vi "Test Read Linker Info.vi"(8 "error in (no error)":errorcluster) -> (0 "error out":errorcluster)   [LabVIEW 2020]
uses:
  classes/Test Runner.Folder/Test Runner.Folder.lvclass
  C:/projects/caraya/src/classes/Test Runner/Test Runner.lvclass
  classes/Test/Test.lvclass
  classes/Assert/Assert.lvclass
  classes/Test Runner/Test Runner.lvclass
panel:
  out "Test VIs":path[](array[path])
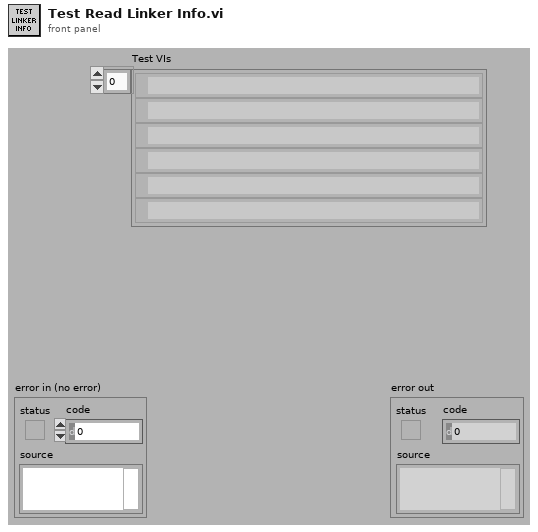
[diagram p1: front panel]
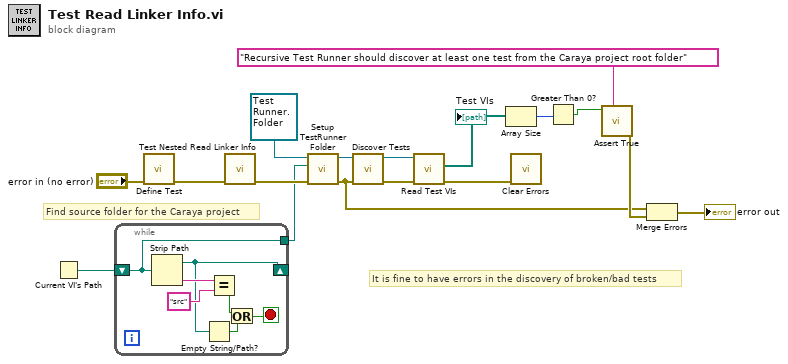
[diagram p0: block diagram]
diagram:
  # "It is fine to have errors in the discovery of broken/bad tests"
  # "Find source folder for the Caraya project"
  n1 = Current VI's Path() -> (path=w7:path)
  n2 = while {
    shift-right: [w18] -> _
    shift-left: w7 -> [w22]
    tunnel: [w22] -> w6
    stop <- w20 stop-if-true
    n3 = Strip Path(path=w22) -> (stripped path=w18:path, name=w24:string)
    n4 = Empty String/Path?(string/path=w18) -> (empty?=w19:bool)
    n5 = Equal?(x=w24, y="src") -> (x = y?=w21:bool)
    n6 = Or(x=w21, y=w19) -> (x .or. y?=w20:bool)
  }
  n7 = call "Define Test.vi"("error in (no error)"="error in (no error)") -> ("error out"=w16:errorcluster)  [unwired: 9 in, 1 out]
  n8 = call "Test Nested Read Linker Info.vi"("error in (no error)"=w16) -> ("error out"=w10:errorcluster)  [unwired: 10 in]
  n9 = call "Setup TestRunner Folder.vi"("error in (no error)"=w10, "Directory to search"=w6, "Test Runner.Folder"=refnum<class "Test Runner.Folder.lvclass"> refnum ("Caraya.lvlib:Test Runner.Folder.lvclass")) -> ("error out"=w2:errorcluster, "Test Runner.Folder out"=w15:refnum<class "Test Runner.Folder.lvclass">)  [unwired: 7 in]
  n10 = call "Discover Tests.vi"("error in (no error)"=w2, "Test Runner in"=w15) -> ("error out"=w8:errorcluster, "Test Runner out"=w9:refnum<class "Test Runner.Folder.lvclass">)  [unwired: 8 in]
  n11 = call "Read Test VIs.vi"("error in (no error)"=w8, "Test Runner in"=w9) -> ("error out"=w4:errorcluster, "Test VIs"=w5:path[])  [unwired: 7 in, 1 out]
  "Test VIs" <- w5
  n12 = Array Size(array=w5) -> (size(s)=w14:i32)
  n13 = call <vilib>:"Clear Errors.vi"("error in (no error)"=w4) -> ()  [unwired: 5 in, 2 out]
  n14 = Greater Than 0?(x=w14) -> (x > 0?=w13:bool)
  n15 = call "Assert True.vi"("Label"="Recursive Test Runner should discover at least one test from the Caraya project root folder", "True?"=w13) -> ("error out"=w3:errorcluster)  [unwired: 8 in, 1 out]
  n16 = Merge Errors(w2, w3) -> (→"error out":errorcluster)
